vi "Get T1T3Window Back.vi"(8 "error in (no error)":errorcluster caption="错误输入（无错误）", 9 "uWindowBack":u32, 10 "nBoard":i32, 11 "nDevId":i32) -> (0 "error out":errorcluster caption="错误输出", 1 "uWindowBack out":u32, 3 "function return":i32)   [LabVIEW 2017, in "smncsftmt.lvlib"]
doc: "__declspec(dllexport) int GetT1T3WindowBack(int nDevId, int nBoard, unsigned int* uWindowBack);"
uses:
  smncsftmt.lvlib
  smncsftmt.dll
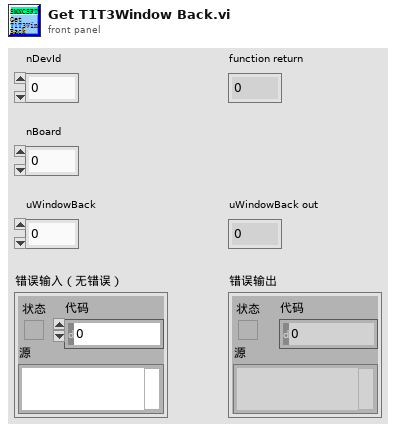
[diagram p1: front panel]
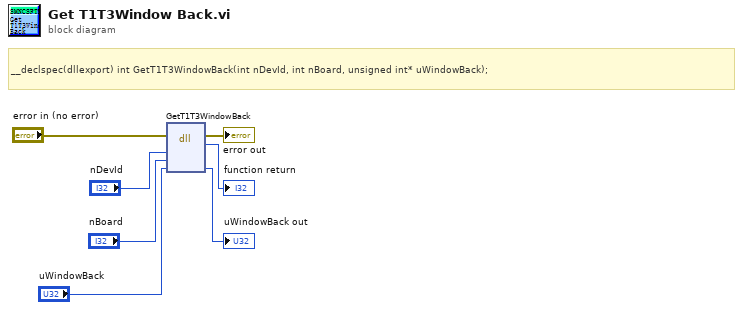
[diagram p0: block diagram]
diagram:
  # "__declspec(dllexport) int GetT1T3WindowBack(int nDevId, int nBoard, unsigned int* uWindowBack);"
  n1 = dll-call lib="PTH2oabs CUsersaDesktop\nLABVIEW范例National InstrumentsLabVIEW 2017user.lib\tsmncsftmtsmncsftmt.*" fn="GetT1T3WindowBack"(error in="error in (no error)", "nDevId"="nDevId", "nBoard"="nBoard", "uWindowBack"="uWindowBack") -> (error out=→"error out":errorcluster, →"function return":i32, "uWindowBack"=→"uWindowBack out":u32)  [unwired: 4 in, 1 out]
